vi "I2C Close.vi"(8 "error in (no error)":errorcluster, 11 "I2C Device":T1) -> (0 "error out":errorcluster)   [LabVIEW 2020, in "wiringPi.lvlib"]
doc: "<b>_______________________________________________________________</b>\n** Author: Juan José Villacorta\n** LabVIEW wrapper for C library <b> wiringPi </b>,\n** https://github.com/WiringPi/WiringPi\n<b>_______________________________________________________________</b>\n/*\n * Close an I2C slave device \n**********************************************************************************\n*/"
uses:
  wiringPi.lvlib
  Type Defs/I2C Device.ctl
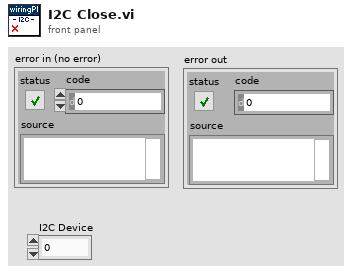
[diagram p1: front panel]
types:
  T1 = typedef "wiringPi.lvlib/I2C Device.ctl" = i32
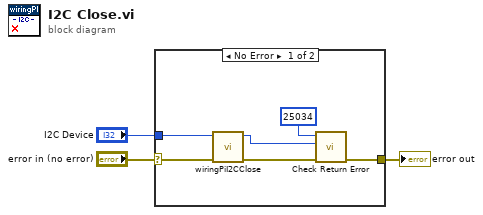
[diagram p0: block diagram]
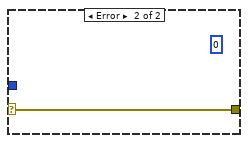
[diagram p2: hidden frame]
diagram:
  n1 = case shown="No Error" "error in (no error)" {
    selector: "error in (no error)" -> [w4 w10]
    tunnel: [w9 w10] -> w2
    tunnel: "I2C Device" -> [w5 _]
    frame No Error {
      n2 = call "wiringPiI2CClose.vi"("error in (no error)"=w4, "devID"=w5) -> ("error out"=w7:errorcluster, "return"=w6:i32)  [unwired: 8 in]
      n3 = call "Check Return Error.vi"("error in (no error)"=w7, "Return code"=w6, "Error number"=25034) -> ("error out"=w9:errorcluster)  [unwired: 8 in]
    }
    frame Error {
      (unwired) 0 ("return")
    }
  }
  "error out" <- w2
